vi "Supported Item Types--constant.vi"() -> (3 "Supported Item Types":string[](array[string]))   [LabVIEW 2020, in "VI Properties Editor.lvlib"]
doc: "Outputs all currently supported file types as reported by the `ProjectItem.TypeString` property node."
uses:
  VI Properties Editor.lvlib
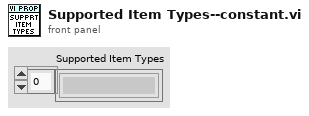
[diagram p1: front panel]
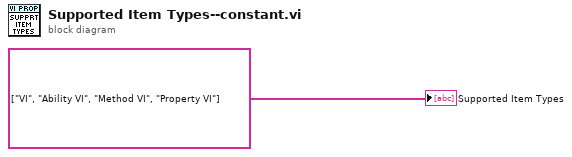
[diagram p0: block diagram]
diagram:
  "Supported Item Types" <- string[] ["VI", "Ability VI", "Method VI", "Property VI"] ("Supported Item Types")
